vi "Configure Sine Generator.vi"(6 "amplitude":dbl=1.0, 7 "frequency":dbl=10.0, 8 "error in":errorcluster, 9 "sample rate":dbl=1000.0, 10 "update interval":u32=100, 11 "number of samples":u32=1000) -> (0 "error out":errorcluster, 3 "generator settings":T1={"Amplitude"=1.0, "Frequency"=10.0, "Sample Rate"=1000.0, "Number of Samples"=1000, "Update Interval ms"=100})   [LabVIEW 2026, in "Sine Generator.lvlib"]
doc: "Configuration stage. Sanitises the user settings so the engine never sees an invalid value: amplitude is made non-negative, sample rate is coerced to 1 S/s .. 10 MS/s, frequency to 0 .. Nyquist (sample rate / 2), number of samples to 2 .. 1 000 000 and update interval to 10 .. 10 000 ms. Returns one generator settings cluster."
uses:
  Sine Generator.lvlib
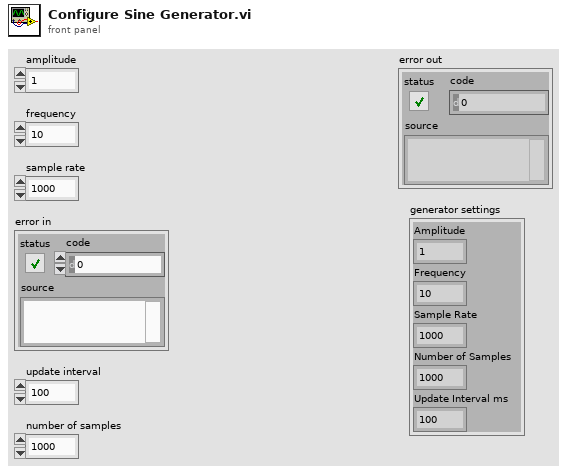
[diagram p1: front panel]
types:
  T1 = cluster{"Amplitude":dbl, "Frequency":dbl, "Sample Rate":dbl, "Number of Samples":i32, "Update Interval ms":i32}
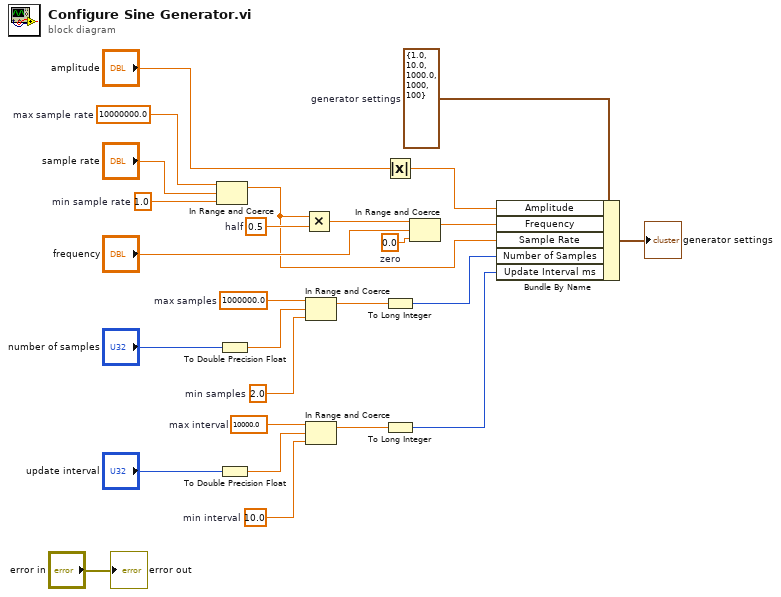
[diagram p0: block diagram]
diagram:
  w3 = T1 {"Amplitude"=1.0, "Frequency"=10.0, "Sample Rate"=1000.0, "Number of Samples"=1000, "Update Interval ms"=100}  # generator settings
  w10 = 10.0  # min interval
  w12 = 10000.0  # max interval
  w15 = 2.0  # min samples
  w17 = 1000000.0  # max samples
  w19 = 0.0  # zero
  w22 = 0.5  # half
  w23 = 1.0  # min sample rate
  w25 = 10000000.0  # max sample rate
  n1 = In Range and Coerce(upper limit=w25, x="sample rate", lower limit=w23) -> (coerced(x)=w6:dbl)  [unwired: 1 out]
  n2 = To Double Precision Float(number="number of samples") -> (double precision float=w16:dbl)
  n3 = To Double Precision Float(number="update interval") -> (double precision float=w11:dbl)
  n4 = Multiply(x=w6, y=w22) -> (x*y=w21:dbl)
  n5 = In Range and Coerce(upper limit=w17, x=w16, lower limit=w15) -> (coerced(x)=w14:dbl)  [unwired: 1 out]
  n6 = In Range and Coerce(upper limit=w12, x=w11, lower limit=w10) -> (coerced(x)=w9:dbl)  [unwired: 1 out]
  n7 = Absolute Value(x="amplitude") -> (abs(x)=w8:dbl)
  n8 = To Long Integer(number=w14) -> (32bit integer=w5:i32)
  n9 = To Long Integer(number=w9) -> (32bit integer=w4:i32)
  n10 = In Range and Coerce(upper limit=w21, x="frequency", lower limit=w19) -> (coerced(x)=w7:dbl)  [unwired: 1 out]
  n11 = Bundle By Name(cluster=w3, "Amplitude"=w8, "Frequency"=w7, "Sample Rate"=w6, "Number of Samples"=w5, "Update Interval ms"=w4) -> (→"generator settings":T1)
  "error out" <- "error in"
